vi "dump data from VIs.vi"(7 "base":path, 8 "error in (no error)":errorcluster, 9 "vi references":refnum<vi>[](array[refnum]), 10 "assets":path, 11 "docs folder":path) -> (0 "error out":errorcluster)   [LabVIEW 2020]
uses:
  <vilib>/JDP Science/JSONtext/LVClass Serializer/JSONtext LVClass Serializer.lvclass
  sphinx terminal direction.ctl
  sphinx terminal data.ctl
  sphinx item data.ctl
  <vilib>/Utility/Data Type/NI_Data Type.lvlib
  41f7d256-710a-436a-832c-a9b2a359d6cb.vi
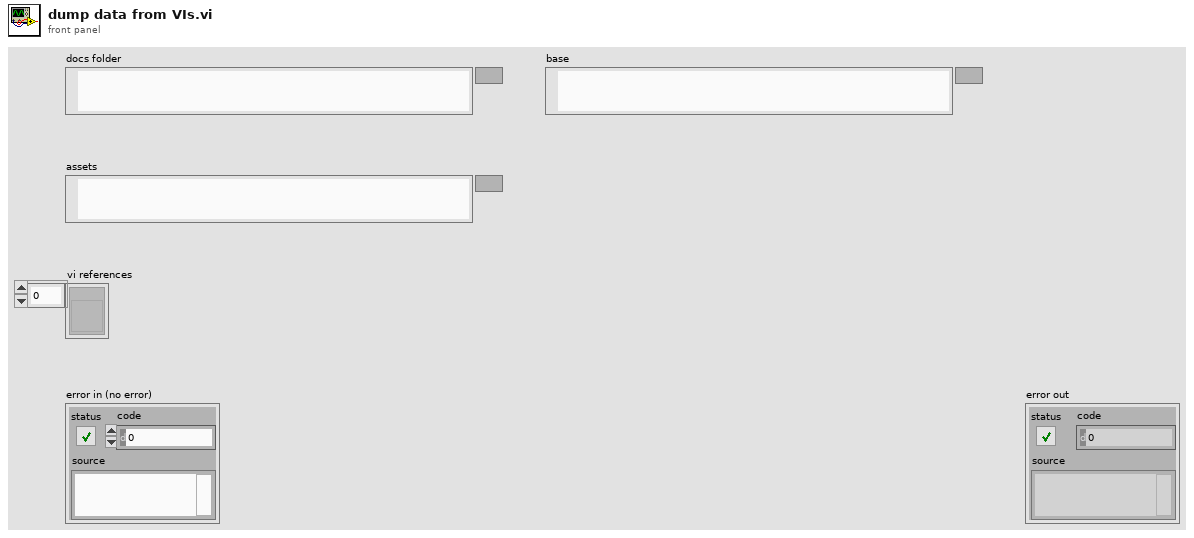
[diagram p1: front panel]
types:
  T1 = typedef "sphinx item data.ctl" = cluster{"id":string, "kind":string, "path":path, "owner":string, "description":string, "icon":path, "terminals":T2[], "relative palette location":string, "connpane":path, "parent ID":string}
  T2 = typedef "sphinx terminal data.ctl" = cluster{"label":string, "direction":T3, "type":string, "type_id":string, "default":string, "description":string, "tip strip":string, "wiring rule":enum16{"Invalid Wire Rule", "Required", "Recommended", "Optional", "Dynamic Dispatch"}, "caption":string}
  T3 = typedef "sphinx terminal direction.ctl" = enum16{"input", "output"}
  T4 = enum16{"open", "replace", "create", "open or create", "replace or create", "replace or create with confirmation"}
  T5 = enum16{"Invalid Wire Rule", "Required", "Recommended", "Optional", "Dynamic Dispatch"}
  T6 = typedef "NI_Data Type.lvlib/Data Type.ctl" = enum8{"Invalid Type", "Void", "I8", "I16", "I32", "I64", "U8", "U16", "U32", "U64", "Single Float", "Double Float", "Extended Float", "Single Complex", "Double Complex", "Extended Complex", "Enum U8", "Enum U16", "Enum U32", "Enum U64", "Single Float With Unit", "Double Float With Unit", "Extended Float With Unit", "Single Complex with Unit", "Double Complex with Unit", "Extended Complex with Unit", "Boolean", "String", "Path", "Picture", "Tag", "Array", "Cluster", "Variant", "LV Variant", "Waveform", "Timestamp", "Digital Waveform", "Digital Data", "ExpressData", "Refnum", "External Data", "VI", "Poly VI", "LabVIEW Class Instance", "Fixed Point", "Set Collection", "Map Collection"}
  T7 = typedef "NI_Data Type.lvlib/Type Definition Info.ctl" = cluster{"Name":string, "Timestamp":u32}
  T8 = typedef "imagedata.ctl" = cluster{"image type":i32, "image depth":i32, "image":u8[], "mask":u8[], "colors":u32[], "Rectangle":cluster{"left":i16, "top":i16, "right":i16, "bottom":i16}}
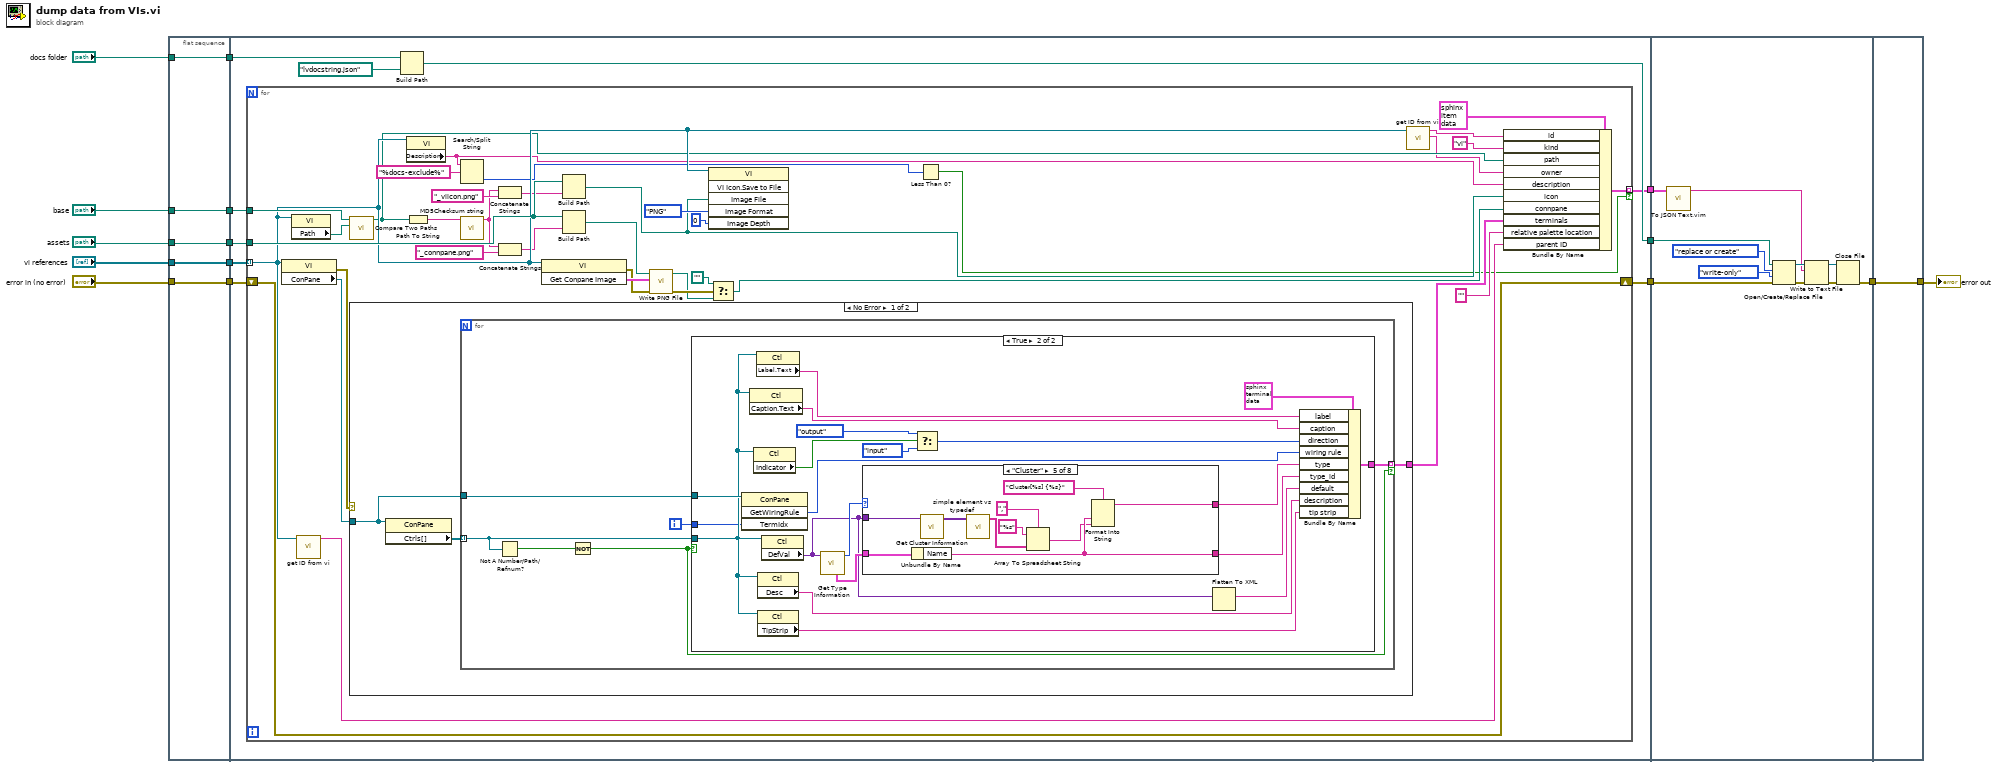
[diagram p0: block diagram]
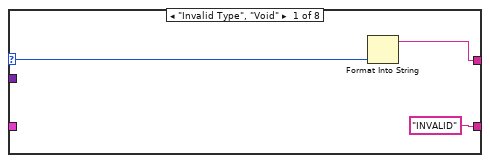
[diagram p3: hidden frame]
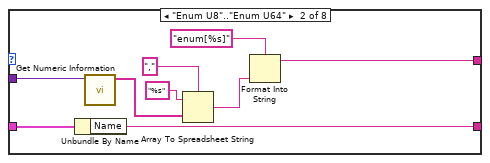
[diagram p4: hidden frame]
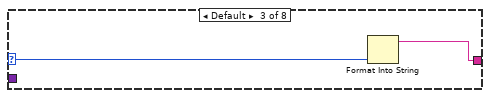
[diagram p5: hidden frame]
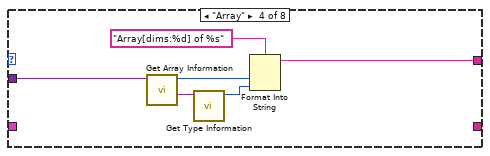
[diagram p6: hidden frame]
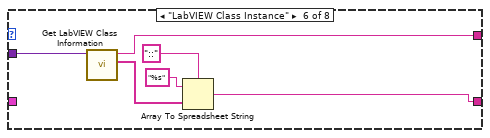
[diagram p7: hidden frame]
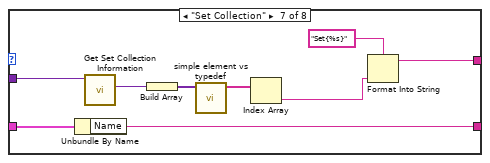
[diagram p8: hidden frame]
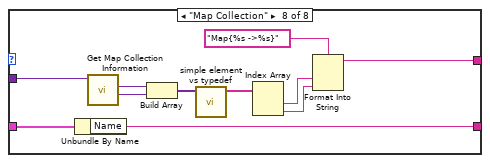
[diagram p9: hidden frame]
diagram:
  n1 = flat-sequence {
    tunnel: "error in (no error)" -> [w18]
    tunnel: "assets" -> [w20]
    tunnel: [w20] -> w15
    tunnel: [w19] -> w14
    tunnel: "docs folder" -> [w19]
    tunnel: [w18] -> w9
    tunnel: "base" -> [w17]
    tunnel: [w17] -> w7
    tunnel: [w16] -> w2
    tunnel: "vi references" -> [w16]
    tunnel: w15 -> [w29]
    tunnel: w14 -> [w28]
    tunnel: w9 -> [w26]
    tunnel: w7 -> [w25]
    tunnel: [w24] -> w5
    tunnel: [w23] -> w4
    tunnel: [w22] -> w3
    tunnel: w2 -> [w21]
    tunnel: [w153] -> w6
    tunnel: w5 -> [w157]
    tunnel: w4 -> [w154]
    tunnel: w3 -> [w152]
    tunnel: [w162] -> w13
    tunnel: w6 -> [w162]
    frame #0 {
    }
    frame #1 {
      n2 = for {
        tunnel: [w30] -> w22 mode=indexing if=w31
        tunnel: w29 -> [w65]
        shift-right: [w64] -> w24
        shift-left: w26 -> [w64]
        tunnel: w25 -> [w63]
        tunnel: w21 -> [w62] mode=indexing
        n3 = property class="VI"(reference=w62) -> (error out=w45:errorcluster, "ConPane"=w46:refnum<vi>)  [unwired: 1 in, 1 out]
        n4 = property class="VI"(reference=w62) -> ("Path"=w39:path)  [unwired: 1 in, 2 out]
        n5 = call "get ID from vi.vi"("VI in"=w62) -> ("VI ID"=w60:string)  [unwired: 9 in, 1 out]
        n6 = call <vilib>:"Compare Two Paths.vi"("Path 2"=w39, "Path 1"=w63) -> ("Relative Path from 1 to 2"=w38:path)  [unwired: 6 in, 3 out]
        n7 = case shown="No Error" w45 {
          tunnel: [w67 _] -> w55
          tunnel: w46 -> [w66 _]
          frame No Error {
            n8 = property class="ConPane"(reference=w66) -> ("Ctrls[]"=w68:refnum<vi>[])  [unwired: 1 in, 2 out]
            n9 = for {
              tunnel: w68 -> [w72] mode=indexing
              tunnel: [w74] -> w67 mode=indexing if=w69
              tunnel: w66 -> [w73]
              i -> [w70]
              n10 = Not A Number/Path/Refnum?(number/path/refnum=w72) -> (NaN/Path/Refnum?=w71:bool)
              n11 = Not(x=w71) -> (.not. x?=w69:bool)
              n12 = case shown="True" w69 {
                tunnel: [_ w93] -> w74
                tunnel: w73 -> [_ w86]
                tunnel: w72 -> [_ w85]
                tunnel: w70 -> [_ w84]
                frame False {
                }
                frame True {
                  n13 = invoke class="ConPane" method="GetWiringRule"(reference=w86, "TermIdx"=w84) -> ("Get Wire Rule"=w83:T5)  [unwired: 2 in, 3 out]
                  n14 = property class="Ctl"(reference=w85) -> ("Caption.Text"=w76:string)  [unwired: 1 in, 2 out]
                  n15 = property class="Ctl"(reference=w85) -> ("Indicator"=w92:bool)  [unwired: 1 in, 2 out]
                  n16 = property class="Ctl"(reference=w85) -> ("Label.Text"=w75:string)  [unwired: 1 in, 2 out]
                  n17 = property class="Ctl"(reference=w85) -> ("Desc"=w87:string)  [unwired: 1 in, 2 out]
                  n18 = property class="Ctl"(reference=w85) -> ("TipStrip"=w88:string)  [unwired: 1 in, 2 out]
                  n19 = property class="Ctl"(reference=w85) -> ("DefVal"=w78:variant)  [unwired: 1 in, 2 out]
                  n20 = call <vilib>:"Get Type Information.vi"("variant"=w78) -> ("type"=w82:T6, "type definition info"=w80:T7)  [unwired: 6 in, 3 out]
                  n21 = case shown="\"Cluster\"" w82 {
                    selector: w82 -> [w95 _ w108 _ _ _ _ _]
                    tunnel: ["INVALID" w105 _ _ w123 w125 w132 w143] -> w81
                    tunnel: w80 -> [_ w106 _ _ w124 _ w133 w144]
                    tunnel: [w96 w99 w107 w109 w116 w129 w134 w145] -> w79
                    tunnel: w78 -> [_ w104 _ w114 w120 w130 w139 w150]
                    frame "Invalid Type", "Void" {
                      n22 = Format Into String(w95) -> (resulting string=w96:string)  [unwired: 3 in, 1 out]
                    }
                    frame "Enum U8".."Enum U64" {
                      n23 = Unbundle By Name(w106) -> ("Name"=w105:string)
                      n24 = call <vilib>:"Get Numeric Information.vi"("variant"=w104) -> ("enum names"=w103:string[])  [unwired: 7 in, 3 out]
                      n25 = Array To Spreadsheet String(delimiter (Tab)=",", array=w103, 3:"%s" ("format string")) -> (spreadsheet string=w102:string)
                      n26 = Format Into String(format string="enum[%s]", w102) -> (resulting string=w99:string)  [unwired: 2 in, 1 out]
                    }
                    frame Default {
                      n27 = Format Into String(w108) -> (resulting string=w107:string)  [unwired: 3 in, 1 out]
                    }
                    frame "Array" {
                      n28 = call <vilib>:"Get Array Information.vi"("variant"=w114) -> ("array element data type"=w111:variant, "number of dimensions"=w112:i32)  [unwired: 7 in, 2 out]
                      n29 = call <vilib>:"Get Type Information.vi"("variant"=w111) -> ("type"=w110:T6)  [unwired: 6 in, 4 out]
                      n30 = Format Into String(format string="Array[dims:%d] of %s", w112, w110) -> (resulting string=w109:string)  [unwired: 2 in, 1 out]
                    }
                    frame "Cluster" {
                      n31 = Unbundle By Name(w124) -> ("Name"=w123:string)
                      n32 = call <vilib>:"Get Cluster Information.vi"("variant"=w120) -> ("cluster elements"=w119:variant[])  [unwired: 9 in, 1 out]
                      n33 = call "simple element vs typedef.vi"("elements"=w119) -> ("simple identifiers"=w118:string[])  [unwired: 10 in]
                      n34 = Array To Spreadsheet String(delimiter (Tab)=",", array=w118, 3:"%s" ("format string")) -> (spreadsheet string=w121:string)
                      n35 = Format Into String(format string="Cluster[%s] {%s}", w123, w121) -> (resulting string=w116:string)  [unwired: 2 in, 1 out]
                    }
                    frame "LabVIEW Class Instance" {
                      n36 = call <vilib>:"Get LabVIEW Class Information.vi"("variant"=w130) -> ("qualified LabVIEW class name"=w126:string[], "LabVIEW class file name"=w129:string)  [unwired: 8 in, 1 out]
                      n37 = Array To Spreadsheet String(delimiter (Tab)="::", array=w126, 3:"%s" ("format string")) -> (spreadsheet string=w125:string)
                    }
                    frame "Set Collection" {
                      n38 = Unbundle By Name(w133) -> ("Name"=w132:string)
                      n39 = call <vilib>:"Get Set Collection Information.vi"("variant"=w139) -> ("element data type"=w138:variant)  [unwired: 9 in, 1 out]
                      n40 = Build Array(w138) -> (w137:variant[])
                      n41 = call "simple element vs typedef.vi"("elements"=w137) -> ("simple identifiers"=w136:string[])  [unwired: 10 in]
                      n42 = Index Array(array=w136) -> (element=w135:string)  [unwired: 1 in]
                      n43 = Format Into String(format string="Set{%s}", w135) -> (resulting string=w134:string)  [unwired: 2 in, 1 out]
                    }
                    frame "Map Collection" {
                      n44 = Unbundle By Name(w144) -> ("Name"=w143:string)
                      n45 = call <vilib>:"Get Map Collection Information.vi"("variant"=w150) -> ("value data type"=w141:variant, "key data type"=w149:variant)  [unwired: 8 in, 1 out]
                      n46 = Build Array(w149, w141) -> (w148:variant[])
                      n47 = call "simple element vs typedef.vi"("elements"=w148) -> ("simple identifiers"=w147:string[])  [unwired: 10 in]
                      n48 = Index Array(array=w147) -> (element #1=w146:string, element #2=w140:string)  [unwired: 2 in]
                      n49 = Format Into String(format string="Map{%s ->%s}", w146, w140) -> (resulting string=w145:string)  [unwired: 2 in, 1 out]
                    }
                  }
                  n50 = Select(t=sphinx_terminal_direction."output" ("direction"), s=w92, f=sphinx_terminal_direction."input" ("direction")) -> (s? t:f=w89:T3)
                  n51 = Flatten To XML(6:w78) -> (2:w77:string)
                  n52 = Bundle By Name(cluster=T2 {"label"="", "direction"=enum."input", "type"="", "type_id"="", "default"="", "description"="", "tip strip"="", "wiring rule"=enum."Invalid Wire Rule", "caption"=""} ("Cluster"), "label"=w75, "caption"=w76, "direction"=w89, "wiring rule"=w83, "type"=w79, "type_id"=w81, "default"=w77, "description"=w87, "tip strip"=w88) -> (w93:T2)
                }
              }
            }
          }
          frame Error {
          }
        }
        n53 = Path To String(path=w38) -> (string=w54:string)
        n54 = property class="VI"(reference=w62) -> ("Description"=w34:string)  [unwired: 1 in, 2 out]
        n55 = Search/Split String(string=w34, search string/char (-)="%docs-exclude%") -> (offset of match=w33:i32)  [unwired: 1 in, 2 out]
        n56 = call <vilib>:"MD5Checksum string.vi"("Message String"=w54) -> ("MD5 message-digest"=w48:string)  [unwired: 10 in]
        n57 = Concatenate Strings(w48, "_viicon.png" ("string")) -> (w52:string)
        n58 = Concatenate Strings(w48, "_connpane.png" ("string")) -> (w51:string)
        n59 = invoke class="VI" method="Get Conpane Image"(reference=w62) -> (error out=w44:errorcluster, "Get Conpane Image"=w57:T8)  [unwired: 2 in, 1 out]
        n60 = Build Path(base path=w65, name or relative path=w52) -> (appended path=w47:path)
        n61 = Build Path(base path=w65, name or relative path=w51) -> (appended path=w49:path)
        n62 = call <vilib>:"Write PNG File.vi"("error in (no error)"=w44, "image data"=w57, "path to PNG file"=w49) -> ("error out"=w43:errorcluster, "path"=w42:path)  [unwired: 7 in]
        n63 = invoke class="VI" method="VI Icon.Save to File"(reference=w62, "Image File"=w47, "Image Format"=enum32{"PNG", "JPEG", "GIF", "BMP"}."PNG", "Image Depth"=0) -> ()  [unwired: 2 in, 6 out]
        n64 = Select(t=path "", s=w43, f=w42) -> (s? t:f=w41:path)
        n65 = Less Than 0?(x=w33) -> (x < 0?=w31:bool)
        n66 = call "get ID from vi.vi"("VI in"=w62) -> ("owning library"=w36:string, "VI ID"=w37:string)  [unwired: 9 in]
        n67 = Bundle By Name(cluster=T1 {"id"="", "kind"="", "path"=path "", "owner"="", "description"="", "icon"=path "", "terminals"=[], "relative palette location"="", "connpane"=path "", "parent ID"=""} ("item"), "id"=w37, "kind"="vi", "path"=w38, "owner"=w36, "description"=w34, "icon"=w47, "connpane"=w41, "terminals"=w55, "relative palette location"="", "parent ID"=w60) -> (w30:T1)
      }
      n68 = Build Path(base path=w28, name or relative path=path "lvdocstring.json") -> (appended path=w23:path)
    }
    frame #2 {
      n69 = call "To JSON Text.vim"("Anything"=w152) -> ("<JSON>"=w151:string)  [unwired: 9 in, 1 out]
      n70 = Open/Create/Replace File(file path (use dialog)=w154, error in=w157, operation (0:open)=T4."replace or create", access (0:read/write)=enum16{"read/write", "read-only", "write-only"}."write-only") -> (refnum out=w158:refnum<file>, error out=w159:errorcluster)  [unwired: 2 in, 1 out]
      n71 = Write to Text File(file (use dialog)=w158, text=w151, error in=w159) -> (refnum out=w160:refnum<file>, error out=w161:errorcluster)  [unwired: 1 in, 1 out]
      n72 = Close File(refnum=w160, error in=w161) -> (error out=w153:errorcluster)  [unwired: 1 out]
    }
    frame #3 {
    }
  }
  "error out" <- w13
